vi "Send Harmonic Response.vi"(7 "id":string, 8 "error in (no error)":errorcluster caption="에러 입력(에러 없음)", 9 "Frequency":dbl[](array[numeric]), 10 "Amplitude":dbl[](array[numeric]), 11 "Instrument Manager 입력":refnum<class "Instrument Manager.lvclass">) -> (0 "error out":errorcluster caption="에러 출력", 3 "Instrument Manager 출력":refnum<class "Instrument Manager.lvclass">)   [LabVIEW 2023, in "Instrument Manager.lvclass"]
uses:
  Instrument Manager.lvclass
  Harmonice Response.ctl
  Instrument Manager.lvclass/Instrument Manager.ctl
  Error Response.ctl
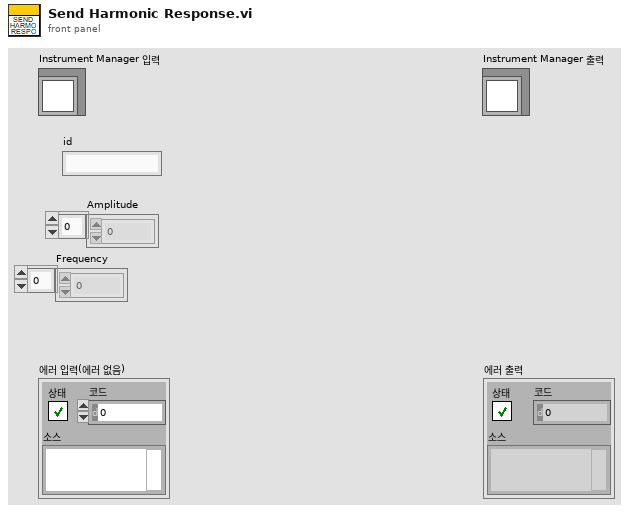
[diagram p1: front panel]
types:
  T1 = typedef "Instrument Manager.lvclass/Harmonice Response.ctl" = cluster{"type":string, "id":string, "status":string, "Result":cluster{"Amplitude":dbl[], "Frequency":dbl[]}}
  T2 = cluster{"Reader Q":refnum<queue>, "Writer Q":refnum<queue>}
  T3 = typedef "Instrument Manager.lvclass/Error Response.ctl" = cluster{"type":string, "id":string, "status":string, "error out":errorcluster}
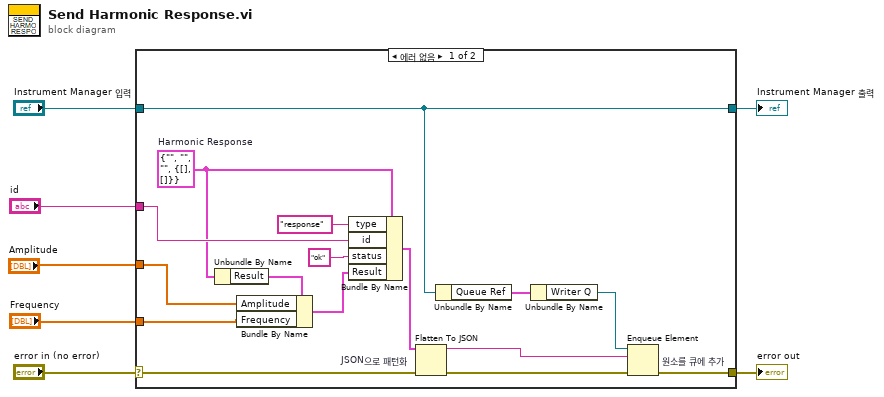
[diagram p0: block diagram]
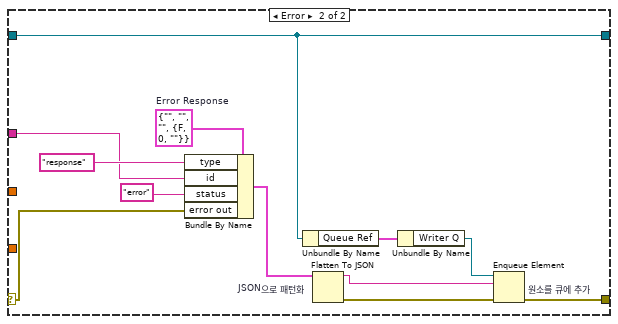
[diagram p2: hidden frame]
diagram:
  n1 = case shown="에러 없음" "error in (no error)" {
    selector: "error in (no error)" -> [w9 w29]
    tunnel: [w13 w28] -> w6
    tunnel: [w10 w24] -> w4
    tunnel: "Instrument Manager 입력" -> [w10 w24]
    tunnel: "id" -> [w23 w27]
    tunnel: "Amplitude" -> [w12 _]
    tunnel: "Frequency" -> [w8 _]
    frame No Error {
      w20 = T1 {"type"="", "id"="", "status"="", "Result"={"Amplitude"=[], "Frequency"=[]}}  # Harmonic Response
      n2 = Unbundle By Name(w20) -> ("Result"=w19:cluster{"Amplitude":dbl[], "Frequency":dbl[]})
      n3 = Bundle By Name(cluster=w19, "Amplitude"=w12, "Frequency"=w8) -> (w18:cluster{"Amplitude":dbl[], "Frequency":dbl[]})
      n4 = Bundle By Name(cluster=w20, "type"="response", "id"=w23, "status"="ok", "Result"=w18) -> (w11:T1)
      n5 = Flatten To JSON "JSON으로 패턴화"(anything=w11, error in (no error)=w9) -> (JSON string=w14:string, 11:w16:errorcluster)  [unwired: 1 in]
      n6 = Unbundle By Name(w10) -> ("Queue Ref"=w17:T2)
      n7 = Unbundle By Name(w17) -> ("Writer Q"=w15:refnum<queue>)
      n8 = Enqueue Element "원소를 큐에 추가"(queue=w15, element=w14, error in (no error)=w16) -> (error out=w13:errorcluster)  [unwired: 1 in, 2 out]
    }
    frame Error {
      w35 = T3 {"type"="", "id"="", "status"="", "error out"={"status"=FALSE, "code"=0, "source"=""}}  # Error Response
      n9 = Bundle By Name(cluster=w35, "type"="response", "id"=w27, "status"="error", "error out"=w29) -> (w31:T3)
      n10 = Unbundle By Name(w24) -> ("Queue Ref"=w25:T2)
      n11 = Flatten To JSON "JSON으로 패턴화"(anything=w31) -> (JSON string=w34:string, 11:w30:errorcluster)  [unwired: 2 in]
      n12 = Unbundle By Name(w25) -> ("Writer Q"=w26:refnum<queue>)
      n13 = Enqueue Element "원소를 큐에 추가"(queue=w26, element=w34, error in (no error)=w30) -> (error out=w28:errorcluster)  [unwired: 1 in, 2 out]
    }
  }
  "error out" <- w6
  "Instrument Manager 출력" <- w4
